vi "Watchdog Whack.vi"(4 "error in (no error)":errorcluster, 5 "reset watchdog after expire? (F)":bool, 7 "watchdogID in":u64) -> (0 "error out":errorcluster, 1 "watchdog status":T1, 3 "watchdogID out":u64)   [LabVIEW 2025]
doc: "<p>Resets the <a href=\"nihelplauncher://docs/csh?context=lvrt_lvrtconcepts_rt_watchdog\">watchdog counter</a> to the value you specify using either the Watchdog Configure VI or the Watchdog Set Attribute VI.</p>"
uses:
  Watchdog status enum.ctl
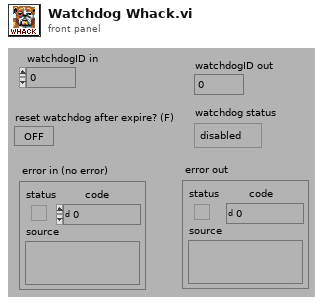
[diagram p1: front panel]
types:
  T1 = typedef "Watchdog status enum.ctl" = enum16{"disabled", "expired", "running"}
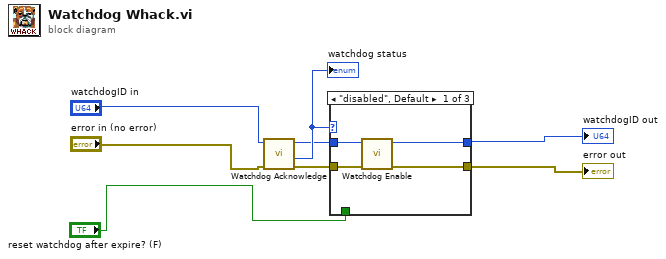
[diagram p0: block diagram]
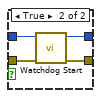
[diagram p3: hidden frame]
diagram:
  n1 = call "Watchdog Acknowledge.vi"("error in (no error)"="error in (no error)", "watchdogID in"="watchdogID in") -> ("error out"=w6:errorcluster, "watchdog status"=w8:T1, "watchdogID out"=w7:u64)  [unwired: 3 in]
  "watchdog status" <- w8
  n2 = case shown="\"disabled\", Default" w8 {
    tunnel: w7 -> [w11 w16 w24]
    tunnel: w6 -> [w12 w17 w25]
    tunnel: [w9 w15 w25] -> w1
    tunnel: [w10 w14 w24] -> w2
    tunnel: "reset watchdog after expire? (F)" -> [_ w13 _]
    frame "disabled", Default {
      n3 = call "Watchdog Enable.vi"("error in (no error)"=w12, "watchdogID in"=w11) -> ("error out"=w9:errorcluster, "watchdogID out"=w10:u64)  [unwired: 4 in]
    }
    frame "expired" {
      n4 = case shown="False" w13 {
        tunnel: w17 -> [w18 w23]
        tunnel: w16 -> [w19 w22]
        tunnel: [w18 w21] -> w15
        tunnel: [w19 w20] -> w14
        frame False {
        }
        frame True {
          n5 = call "Watchdog Start.vi"("error in (no error)"=w23, "watchdogID in"=w22) -> ("error out"=w21:errorcluster, "watchdogID out"=w20:u64)  [unwired: 4 in]
        }
      }
    }
    frame "running" {
    }
  }
  "watchdogID out" <- w2
  "error out" <- w1
